vi "CmdCtl Immed Completion Checki.vi"(7 "timeout (ms)":u32=50, 9 "Start Time (ms)":u32, 11 "current time (ms)":u32) -> (3 "Completion":T1)   [LabVIEW 2023]
uses:
  <vilib>/MRC/Types/CmdCtl Completion.ctl
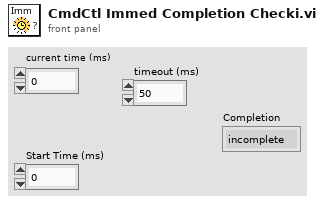
[diagram p1: front panel]
types:
  T1 = typedef "CmdCtl Completion.ctl" = enum16{"incomplete", "finished"}
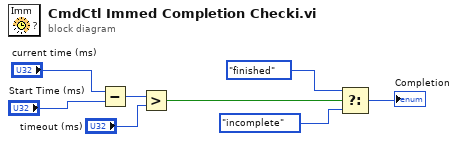
[diagram p0: block diagram]
diagram:
  n1 = Subtract(x="current time (ms)", y="Start Time (ms)") -> (x-y=w6:u32)
  n2 = Greater?(x=w6, y="timeout (ms)") -> (0:w1:bool)
  n3 = Select(t=CmdCtl_Completion."finished", s=w1, f=CmdCtl_Completion."incomplete") -> (s? t:f=→"Completion":T1)
